vi "Prcess Data.vi"(8 "error in (no error)":errorcluster, 9 "Running":refnum<vi>, 10 "XY Plot":refnum<vi>, 11 "Leakage":refnum<class "Leakage.lvclass">) -> (0 "error out":errorcluster, 3 "Leakage out":refnum<class "Leakage.lvclass">)   [LabVIEW 2025, in "Flow Grind.lvlib" / "Leakage.lvclass"]
uses:
  Leakage.lvclass
  Leakage.lvclass/Leakage.ctl
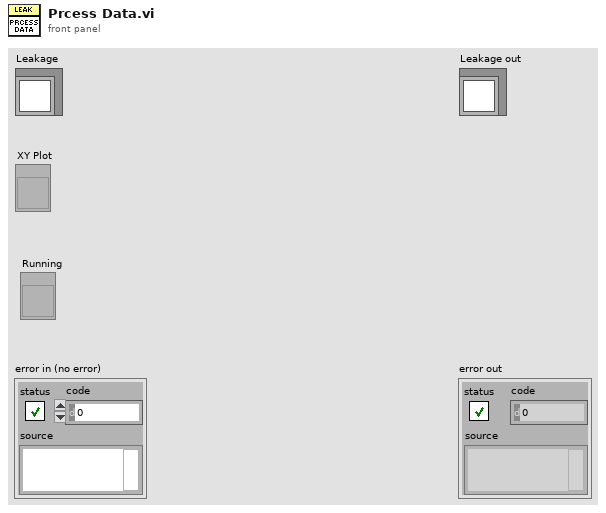
[diagram p1: front panel]
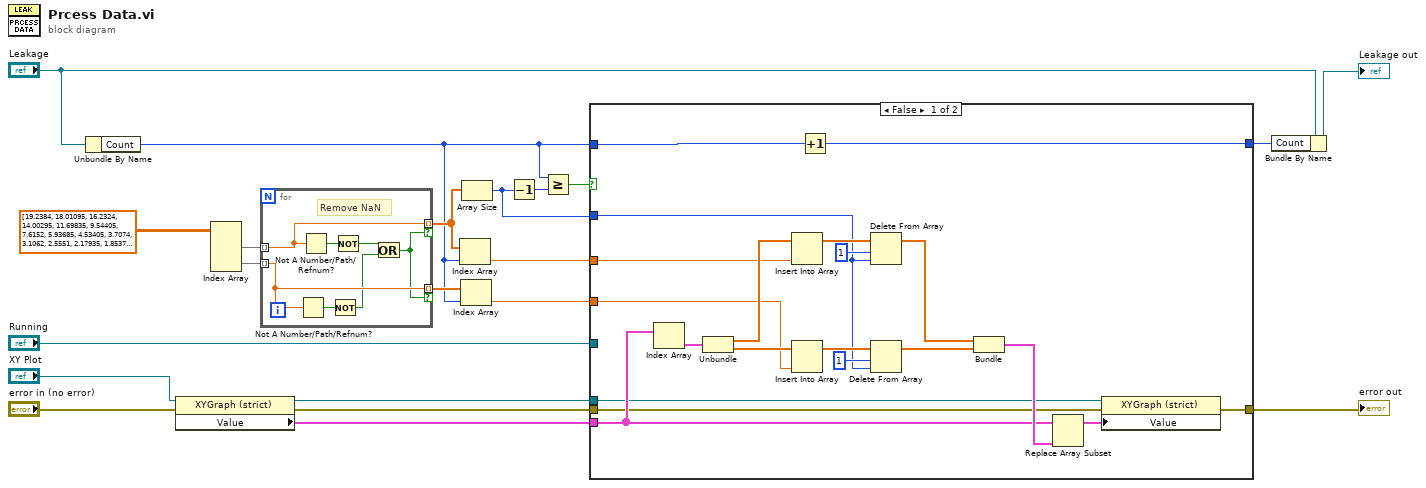
[diagram p0: block diagram]
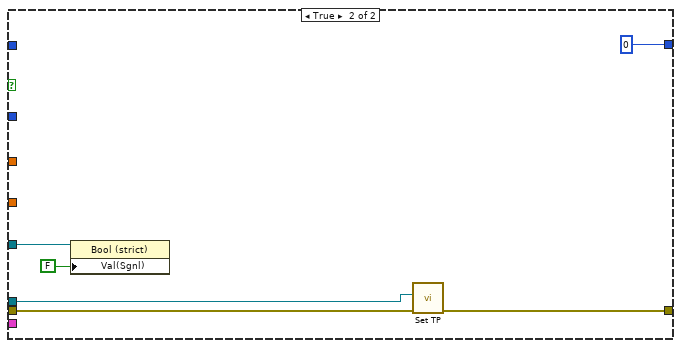
[diagram p2: hidden frame]
diagram:
  n1 = Unbundle By Name("Leakage") -> ("Count"=w7:i32)
  n2 = property class="XYGraph (strict)"(reference="XY Plot", error in="error in (no error)") -> (reference out=w8:refnum<vi>, error out=w12:errorcluster, "Value"=w11:cluster{dbl[], dbl[]}[])
  n3 = Index Array(array=dbl[][] [[19.2384, 18.01095, 16.2324, 14.00295, 11.69835, 9.54405, 7.6152, 5.93685, 4.53405, 3.7074, 3.1062, 2.5551, 2.17935, 1.8537, 1.52805, 1.12725, 0.8517, 0.5511, 0.2004, -0.0501, -0.27555, -0.501, -0.72645, -1.02705, -1.3026, -1.6032, -2.02905, -2.505, -3.03105, -3.58215, -4.2084, -4.88475, -5.78655, -6.43785, -7.28955, -8.517, -9.79455, -11.1723, -13.20135, -14.8797, -16.6332, -18.3366, nan, nan, nan, nan, nan, nan, nan, nan, nan, nan, nan, nan, nan, nan, nan, nan, nan, nan, nan, nan, nan, nan, nan, nan, nan, nan], [-14.7544019, -14.7521866, -14.750236, -14.7428783, -14.7214317, -14.6706498, -14.6196725, -14.5459192, -14.4738652, -14.4142389, -14.3596933, -14.2987315, -14.2463503, -14.2064567, -14.1571661, -14.1087058, -14.0807395, -14.0370388, -14.0237377, -14.0261081, -14.0226897, -14.0277151, -14.0392527, -14.0496884, -14.0610192, -14.0847393, -14.114795, -14.1626131, -14.2117593, -14.2546388, -14.2988227, -14.3518833, -14.394926, -14.4327158, -14.4763993, -14.5148669, -14.5561009, -14.5969939, -14.6351609, -14.6631068, -14.695462, -14.7129955, nan, nan, nan, nan, nan, nan, nan, nan, nan, nan, nan, nan, nan, nan, nan, nan, nan, nan, nan, nan, nan, nan, nan, nan, nan, nan], [0.0, 0.0, 0.0, 0.0, 0.0, 0.0, 0.0, 0.0, 0.0, 0.0, 0.0, 0.0, 0.0, 0.0, 0.0, 0.0, 0.0, 0.0, 0.0, 0.0, 0.0, 0.0, 0.0, 0.0, 0.0, 0.0, 0.0, 0.0, 0.0, 0.0, 0.0, 0.0, 0.0, 0.0, 0.0, 0.0, 0.0, 0.0, 0.0, 0.0, 0.0, 0.0, 0.0, 0.0, 0.0, 0.0, 0.0, 0.0, 0.0, 0.0, 0.0, 0.0, 0.0, 0.0, 0.0, 0.0, 0.0, 0.0, 0.0, 0.0, 0.0, 0.0, 0.0, 0.0, 0.0, 0.0, 0.0, 0.0], [0.0, 0.0, 0.0, 0.0, 0.0, 0.0, 0.0, 0.0, 0.0, 0.0, 0.0, 0.0, 0.0, 0.0, 0.0, 0.0, 0.0, 0.0, 0.0, 0.0, 0.0, 0.0, 0.0, 0.0, 0.0, 0.0, 0.0, 0.0, 0.0, 0.0, 0.0, 0.0, 0.0, 0.0, 0.0, 0.0, 0.0, 0.0, 0.0, 0.0, 0.0, 0.0, 0.0, 0.0, 0.0, 0.0, 0.0, 0.0, 0.0, 0.0, 0.0, 0.0, 0.0, 0.0, 0.0, 0.0, 0.0, 0.0, 0.0, 0.0, 0.0, 0.0, 0.0, 0.0, 0.0, 0.0, 0.0, 0.0]] ("array1")) -> (element #1=w21:dbl[], element #2=w20:dbl[])  [unwired: 4 in]
  n4 = for {
    tunnel: w21 -> [w28] mode=indexing
    tunnel: w20 -> [w25] mode=indexing
    tunnel: [w28] -> w17 mode=indexing if=w22
    tunnel: [w25] -> w19 mode=indexing if=w22
    # "Remove NaN"
    n5 = Not A Number/Path/Refnum?(number/path/refnum=w25) -> (NaN/Path/Refnum?=w26:bool)
    n6 = Not A Number/Path/Refnum?(number/path/refnum=w28) -> (NaN/Path/Refnum?=w27:bool)
    n7 = Not(x=w26) -> (.not. x?=w24:bool)
    n8 = Not(x=w27) -> (.not. x?=w23:bool)
    n9 = Or(x=w23, y=w24) -> (x .or. y?=w22:bool)
  }
  n10 = Index Array(array=w17, index=w7) -> (element=w15:dbl)
  n11 = Index Array(array=w19, index=w7) -> (element=w3:dbl)
  n12 = Array Size(array=w17) -> (size(s)=w6:i32)
  n13 = Decrement(x=w6) -> (x-1=w18:i32)
  n14 = Greater Or Equal?(x=w7, y=w18) -> (x >= y?=w16:bool)
  n15 = case shown="False" w16 {
    tunnel: w15 -> [w36 _]
    tunnel: w3 -> [w37 _]
    tunnel: w12 -> [w31 w51]
    tunnel: w11 -> [w38 _]
    tunnel: [w35 0] -> w9
    tunnel: w8 -> [w32 w49]
    tunnel: w7 -> [w34 _]
    tunnel: "Running" -> [_ w53]
    tunnel: w6 -> [w33 _]
    tunnel: [w29 w50] -> w5
    frame False {
      n16 = Index Array(array=w38) -> (element=w47:cluster{dbl[], dbl[]})  [unwired: 1 in]
      n17 = Unbundle(w47) -> (w45:dbl[], w46:dbl[])
      n18 = Insert Into Array(array=w45, new element=w36) -> (w42:dbl[])  [unwired: 1 in]
      n19 = Insert Into Array(array=w46, new element=w37) -> (w43:dbl[])  [unwired: 1 in]
      n20 = Increment(x=w34) -> (x+1=w35:i32)
      n21 = Delete From Array(array=w42, length=1, index=w33) -> (array with subset deleted=w40:dbl[])  [unwired: 1 out]
      n22 = Delete From Array(array=w43, length=1, index=w33) -> (array with subset deleted=w39:dbl[])  [unwired: 1 out]
      n23 = Bundle(w40, w39) -> (w48:cluster{dbl[], dbl[]})  [unwired: 1 in]
      n24 = Replace Array Subset(array=w38, new element=w48) -> (w30:cluster{dbl[], dbl[]}[])  [unwired: 1 in]
      n25 = property class="XYGraph (strict)"(reference=w32, error in=w31, "Value"=w30) -> (error out=w29:errorcluster)  [unwired: 1 out]
    }
    frame True {
      n26 = property class="Bool (strict)"(reference=w53, "Val(Sgnl)"=FALSE ("Value (Signaling)")) -> ()  [unwired: 1 in, 2 out]
      n27 = call "Set TP.vi"("error in (no error)"=w51, "Main"=w49) -> ("error out"=w50:errorcluster)  [unwired: 9 in]
    }
  }
  "error out" <- w5
  n28 = Bundle By Name(cluster="Leakage", "Count"=w9) -> (→"Leakage out":refnum<class "Leakage.lvclass">)
